vi "test_lidar.vi"() -> ()   [LabVIEW 2017]
panel:
  out "Data":cluster{"Angle":dbl, dbl}[](array[cluster])
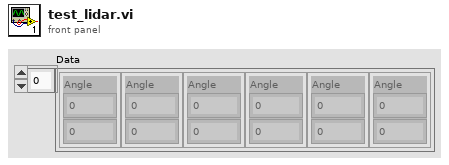
[diagram p1: front panel]
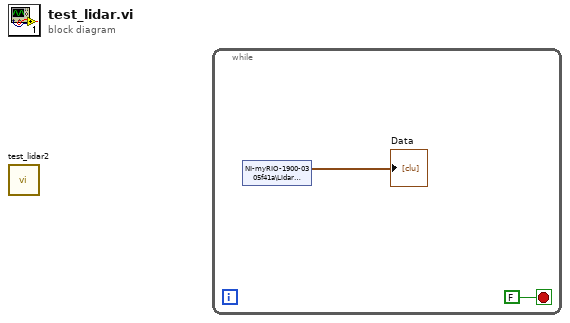
[diagram p0: block diagram]
diagram:
  n1 = call "test_lidar2.vi"() -> ()  [unwired: 12 in]
  n2 = while {
    stop <- FALSE stop-if-true
    n3 = shared-variable "NI-myRIO-1900-0305f41a\\Lidar Library.lvlib\\Data"() -> (→"Data":cluster{"Angle":dbl, dbl}[])  [unwired: 1 in, 1 out]
  }
